vi "PatchCore_DS_Reader.vi"(4 "Read Options":T1={"Read Bads?"=TRUE, "Read GTs?"=TRUE, "Update. DS Stats?"=FALSE}, 6 "Good Unique Labels":string[](array[string])=["normal", "good", "OK"], 7 "PreProc_Options_in":T2={"DS_Name"="", "Input_Dims"={"C"=3, "H"=224, "W"=224}, "Cropping"={"Left"=0.0, "Top"=0.0, "Right"=1.0, "Bottom"=1.0}, "Interpolation Type"=1, "MultiStage_ReSample?"=TRUE, "Dataset_Stats"={"means"={"R"=0.19849297, "G"=0.18453708, "B"=0.19229858}, "stds"={"R"=0.22779399, "G"=0.21340185, "B"=0.19371489}}} {"Dataset_Stats"."stds"."R" format="%#_3g"; "Dataset_Stats"."stds"."G" format="%#_3g"; "Dataset_Stats"."stds"."B" format="%#_3g"; "Dataset_Stats"."means"."R" format="%#_3g"; "Dataset_Stats"."means"."G" format="%#_3g"; "Dataset_Stats"."means"."B" format="%#_3g"; "Interpolation Type" items=["Zero Order", "Bi-Linear", "Quadratic", "Cubic Spline"]}, 8 "error in":errorcluster, 10 "GT Folder Path":path, 11 "Folder Path":path) -> (0 "error out":errorcluster, 1 "PreProc_Options_out":T2={"DS_Name"="", "Input_Dims"={"C"=3, "H"=224, "W"=224}, "Cropping"={"Left"=0.0, "Top"=0.0, "Right"=1.0, "Bottom"=1.0}, "Interpolation Type"=1, "MultiStage_ReSample?"=TRUE, "Dataset_Stats"={"means"={"R"=0.19849297, "G"=0.18453708, "B"=0.19229858}, "stds"={"R"=0.22779399, "G"=0.21340185, "B"=0.19371489}}} {"Dataset_Stats"."stds"."R" format="%#_3g"; "Dataset_Stats"."stds"."G" format="%#_3g"; "Dataset_Stats"."stds"."B" format="%#_3g"; "Dataset_Stats"."means"."R" format="%#_3g"; "Dataset_Stats"."means"."G" format="%#_3g"; "Dataset_Stats"."means"."B" format="%#_3g"; "Interpolation Type" items=["Zero Order", "Bi-Linear", "Quadratic", "Cubic Spline"]}, 3 "Dataset":T7, 5 "dT_DS_Reader":dbl=1.5722605000046315)   [LabVIEW 2020]
uses:
  <vilib>/Ngene/Deep Learning Toolkit/Toolkit/NN_Data/API/DataSet/DataSet_Types/NN_DataSet(In3D_Out3D).ctl
  <vilib>/Ngene/Deep Learning Toolkit/Toolkit/NN_Data/API/NN_Dims(C,H,W).ctl
  <vilib>/Ngene/Deep Learning Toolkit/Toolkit/NN_Data/Controls/DataRef_Types/4D/NN_Data_ref(4D_SGL).ctl
  <vilib>/Ngene/DeepLTK Anomaly Detection Addon/Toolkit/API/Controls/NNPC_PreProcessing_Options.ctl
  <vilib>/Ngene/DeepLTK Anomaly Detection Addon/Toolkit/API/Controls/Crop_CFG.ctl
  <vilib>/Ngene/DeepLTK Anomaly Detection Addon/Toolkit/API/Controls/NNPC_DS_Stats.ctl
  <vilib>/Ngene/DeepLTK Anomaly Detection Addon/Toolkit/API/Controls/Image_Stats_RGB.ctl
  Controls/Read_Options.ctl
  <vilib>/Ngene/DeepLTK Anomaly Detection Addon/Toolkit/API/Controls/NNPC_DS_Custom_Data.ctl
  99e5ce4f-b18a-48c0-8340-627915dc1de5.vi
  39b6eea5-2cfc-4ae9-b230-8dd7afd04afa.vi
  <vilib>/Utility/High Resolution Relative Seconds.vi
  <vilib>/Ngene/Deep Learning Toolkit/Toolkit/Deep_Learning_Toolkit_by_Ngene.lvlib
  <vilib>/Ngene/DeepLTK Anomaly Detection Addon/Toolkit/DeepLTK_Anomaly_Detection_Addon.lvlib
  <vilib>/vision/NI_Vision_Development_Module.lvlib
panel:
  out "Progress":i32=41
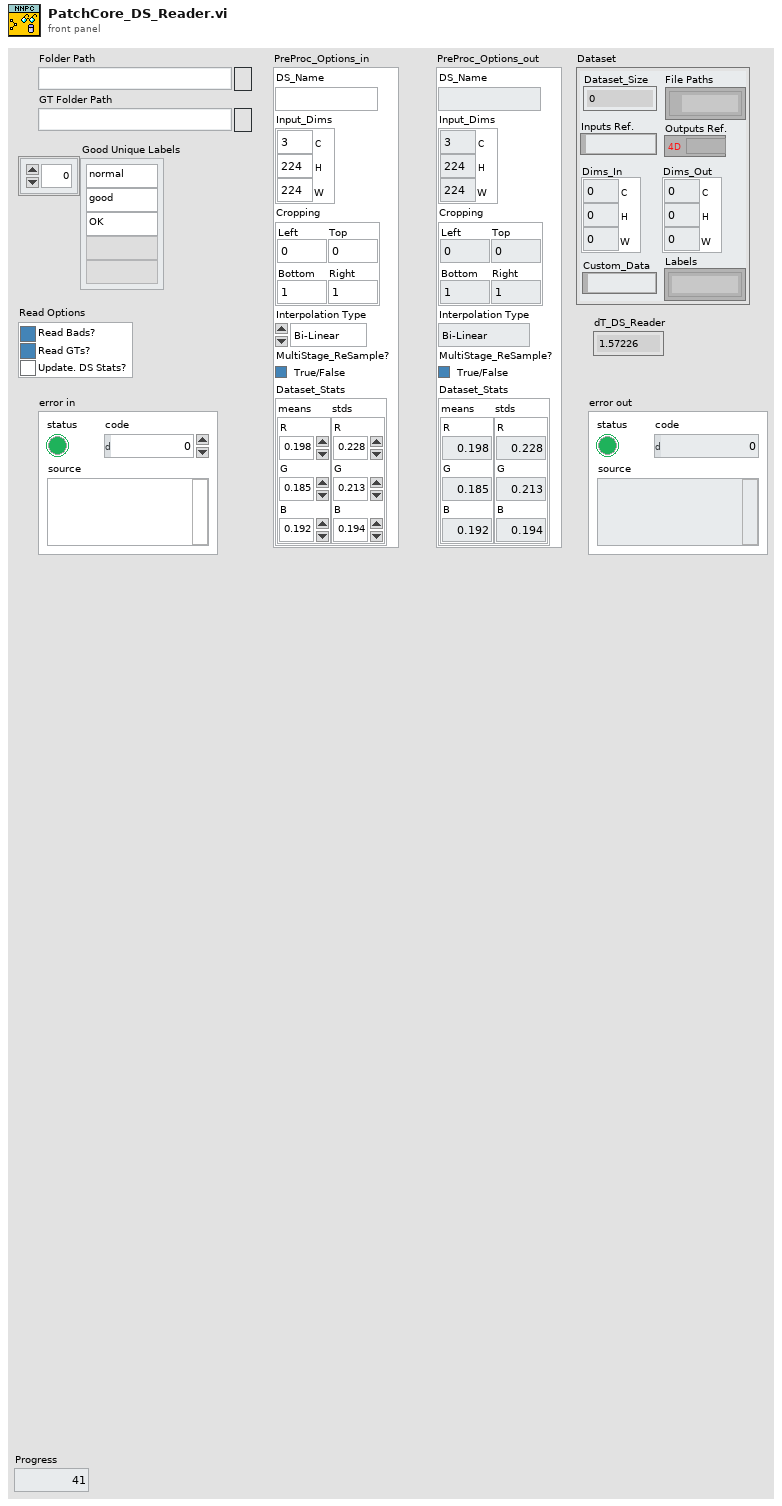
[diagram p1: front panel]
types:
  T1 = typedef "Read_Options.ctl" = cluster{"Read Bads?":bool, "Read GTs?":bool, "Update. DS Stats?":bool}
  T2 = typedef "DeepLTK_Anomaly_Detection_Addon.lvlib/NNPC_PreProcessing_Options.ctl" = cluster{"DS_Name":string, "Input_Dims":T3, "Cropping":T4, "Interpolation Type":u32, "MultiStage_ReSample?":bool, "Dataset_Stats":T5}
  T3 = typedef "Deep_Learning_Toolkit_by_Ngene.lvlib/NN_Dims(C,H,W).ctl" = cluster{"C":i32, "H":i32, "W":i32}
  T4 = typedef "DeepLTK_Anomaly_Detection_Addon.lvlib/Crop_CFG.ctl" = cluster{"Left":sgl, "Top":sgl, "Right":sgl, "Bottom":sgl}
  T5 = typedef "DeepLTK_Anomaly_Detection_Addon.lvlib/NNPC_DS_Stats.ctl" = cluster{"means":T6, "stds":T6}
  T6 = typedef "DeepLTK_Anomaly_Detection_Addon.lvlib/Image_Stats_RGB.ctl" = cluster{"R":sgl, "G":sgl, "B":sgl}
  T7 = typedef "Deep_Learning_Toolkit_by_Ngene.lvlib/NN_DataSet(In3D_Out3D).ctl" = cluster{"Dataset_Size":i32, "Dims_In":T3, "Labels":string[], "File Paths":path[], "Outputs Ref.":T8, "Inputs Ref.":variant, "Dims_Out":T3, "Custom_Data":variant}
  T8 = typedef "Deep_Learning_Toolkit_by_Ngene.lvlib/NN_Data_ref(4D_SGL).ctl" = refnum<data-value>
  T9 = typedef "DeepLTK_Anomaly_Detection_Addon.lvlib/NNPC_DS_Custom_Data.ctl" = cluster{"HasPixelGT?":bool, "ImageGT":refnum<data-value>, "PixelGT":refnum<data-value>}
  T10 = typedef "Image Type" = u32
  T11 = typedef "IMAQ Image.ctl" = refnum<image>
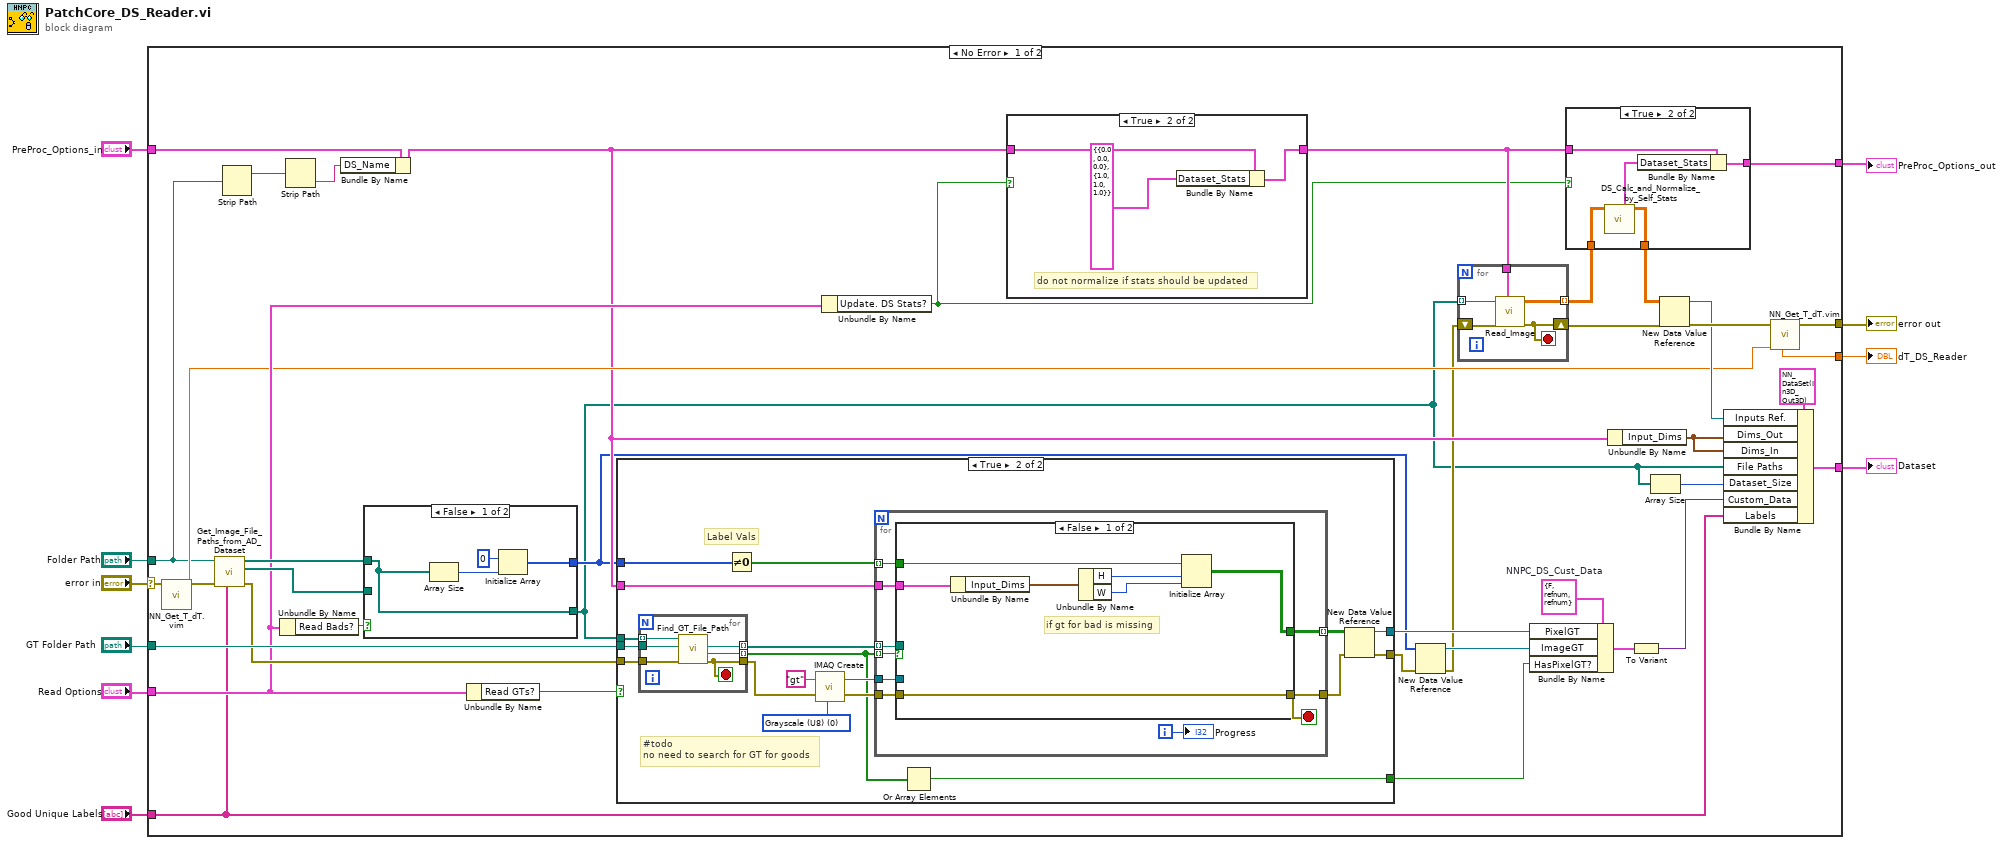
[diagram p0: block diagram]
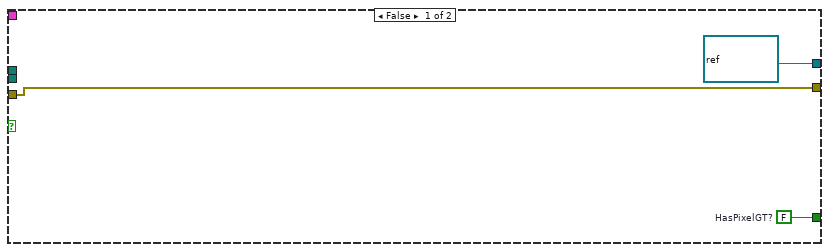
[diagram p2: hidden frame]
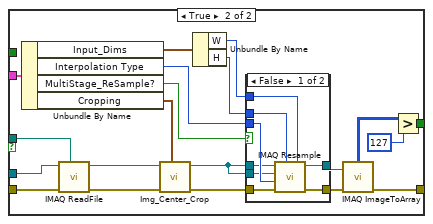
[diagram p3: hidden frame]
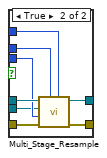
[diagram p4: hidden frame]
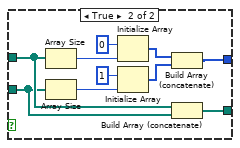
[diagram p5: hidden frame]
diagram:
  n1 = case shown="No Error" "error in" {
    selector: "error in" -> [w50 w160]
    tunnel: [w49 _] -> w9
    tunnel: "GT Folder Path" -> [w47 _]
    tunnel: "Good Unique Labels" -> [w19 _]
    tunnel: "Read Options" -> [w40 _]
    tunnel: [w37 w160] -> w5
    tunnel: [w35 _] -> w4
    tunnel: "Folder Path" -> [w34 _]
    tunnel: "PreProc_Options_in" -> [w31 _]
    tunnel: [w23 _] -> w1
    frame No Error {
      w22 = T9 {"HasPixelGT?"=FALSE, "ImageGT"=refnum, "PixelGT"=refnum}  # NNPC_DS_Cust_Data
      n2 = call "NN_Get_T_dT.vim"("error in"=w50) -> ("T_out"=w36:dbl, "error out"=w38:errorcluster)  [unwired: 6 in, 1 out]
      n3 = call "Get_Image_File_Paths_from_AD_Dataset.vi"("Good Folder Names"=w19, "error in"=w38, "Dataset Folder"=w34) -> ("error out"=w42:errorcluster, "Bad Dataset Files"=w45:path[], "Good Dataset Files"=w44:path[])  [unwired: 6 in]
      n4 = Strip Path(path=w34) -> (stripped path=w33:path)  [unwired: 1 out]
      n5 = Unbundle By Name(w40) -> ("Read Bads?"=w43:bool)
      n6 = Strip Path(path=w33) -> (name=w29:string)  [unwired: 1 out]
      n7 = Bundle By Name(cluster=w31, "DS_Name"=w29) -> (w30:T2)
      n8 = case shown="False" w43 {
        tunnel: w44 -> [w131 w142]
        tunnel: [w131 w143] -> w12
        tunnel: w45 -> [_ w137]
        tunnel: [w130 w134] -> w16
        frame False {
          n9 = Array Size(array=w131) -> (size(s)=w133:i32)
          n10 = Initialize Array(0 ("element"), w133) -> (w130:i32[])
        }
        frame True {
          n11 = Array Size(array=w142) -> (size(s)=w141:i32)
          n12 = Array Size(array=w137) -> (size(s)=w138:i32)
          n13 = Initialize Array(0 ("element"), w141) -> (w136:i32[])
          n14 = Initialize Array(1 ("element"), w138) -> (w135:i32[])
          n15 = Build Array (concatenate)(w136, w135) -> (w134:i32[])
          n16 = Build Array (concatenate)(w142, w137) -> (w143:path[])
        }
      }
      n17 = Unbundle By Name(w40) -> ("Read GTs?"=w20:bool)
      n18 = case shown="True" w20 {
        tunnel: w42 -> [w53 w64]
        tunnel: w47 -> [_ w66]
        tunnel: [w53 w54] -> w14
        tunnel: w12 -> [_ w65]
        tunnel: w16 -> [_ w59]
        tunnel: w30 -> [_ w62]
        tunnel: [refnum<data-value> refnum ("data value reference") w60] -> w17
        tunnel: [w51 w56] -> w11
        frame False {
          w51 = FALSE  # HasPixelGT?
        }
        frame True {
          w68 = T10 0 items=["Grayscale (U8)", "Grayscale (I16)", "Grayscale (SGL)", "Complex (CSG)", "RGB (U32)", "HSL (U32)", "RGB (U64)", "Grayscale (U16)"] ("Image Type")
          # "#todo\nno need to search for GT for goods"
          # "Label Vals"
          n19 = for {
            tunnel: w66 -> [w77]
            tunnel: w65 -> [w74] mode=indexing
            tunnel: [w75] -> w67 mode=indexing
            tunnel: [w76] -> w57 mode=indexing
            tunnel: w64 -> [w73]
            tunnel: [w72] -> w63
            stop <- w72 stop-if-true
            n20 = call "Find_GT_File_Path.vi"("error in"=w73, "GT Mask Folder Path"=w77, "Image File Path"=w74) -> ("error out"=w72:errorcluster, "Found?"=w76:bool, "GT File Path"=w75:path)  [unwired: 5 in, 1 out]
          }
          n21 = Not Equal To 0?(x=w59) -> (x != 0?=w58:bool[])
          n22 = call "IMAQ Create"("Image Name"="gt", "Image Type"=w68, "error in (no error)"=w63) -> ("New Image"=w71:T11, "error out"=w69:errorcluster)  [unwired: 2 in]
          n23 = for {
            tunnel: w71 -> [w86]
            tunnel: w67 -> [w84] mode=indexing
            tunnel: w57 -> [w81] mode=indexing
            tunnel: w58 -> [w80] mode=indexing
            tunnel: w62 -> [w79]
            tunnel: [w78] -> w61 mode=indexing
            tunnel: w69 -> [w85]
            tunnel: [w82] -> w55
            i -> [w83]
            stop <- w82 stop-if-true
            n24 = case shown="False" w81 {
              tunnel: w86 -> [_ w113]
              tunnel: w85 -> [w93 w112]
              tunnel: w84 -> [_ w111]
              tunnel: [w93 w110] -> w82
              tunnel: w80 -> [w90 _]
              tunnel: w79 -> [w88 w108]
              tunnel: [w87 w105] -> w78
              frame False {
                # "if gt for bad is missing"
                n25 = Unbundle By Name(w88) -> ("Input_Dims"=w89:T3)
                n26 = Unbundle By Name(w89) -> ("H"=w91:i32, "W"=w92:i32)
                n27 = Initialize Array(w90, w91, w92) -> (w87:bool[][])
              }
              frame True {
                n28 = Unbundle By Name(w108) -> ("Input_Dims"=w109:T3, "Interpolation Type"=w99:u32, "MultiStage_ReSample?"=w98:bool, "Cropping"=w102:T4)
                n29 = call "IMAQ ReadFile"("File Path"=w111, "error in (no error)"=w112, "Image"=w113) -> ("error out"=w103:errorcluster, "Image Out"=w104:T11)  [unwired: 4 in, 3 out]
                n30 = call "Img_Center_Crop.vi"("Crop_CFG"=w102, "error in"=w103, "Image Src In"=w104) -> ("error out"=w95:errorcluster, "Image Dest Out"=w94:T11)  [unwired: 7 in]
                n31 = Unbundle By Name(w109) -> ("W"=w100:i32, "H"=w101:i32)
                n32 = case shown="False" w98 {
                  tunnel: [w121 w126] -> w96
                  tunnel: [w120 w127] -> w97
                  tunnel: w99 -> [w119 w123]
                  tunnel: w94 -> [w115 w124]
                  tunnel: w100 -> [w118 w125]
                  tunnel: w101 -> [w117 w128]
                  tunnel: w95 -> [w116 w129]
                  tunnel: w94 -> [w114 w122]
                  frame False {
                    n33 = call "IMAQ Resample"("X Resolution"=w118, "Y Resolution"=w117, "error in (no error)"=w116, "Interpolation Type"=w119, "Image Dst"=w114, "Image Src"=w115) -> ("error out"=w121:errorcluster, "Image Dst Out"=w120:T11)  [unwired: 4 in]
                  }
                  frame True {
                    n34 = call "Multi_Stage_Resample.vi"("X Resolution"=w125, "Y Resolution"=w128, "error in"=w129, "Interpolation Type"=w123, "Image Dest In"=w122, "Image Src"=w124) -> ("error out"=w126:errorcluster, "Img out"=w127:T11)  [unwired: 4 in]
                  }
                }
                n35 = call "IMAQ ImageToArray"("error in (no error)"=w96, "Image"=w97) -> ("error out"=w110:errorcluster, "Image Pixels (U8)"=w107:u8[][])  [unwired: 2 in, 3 out]
                n36 = Greater?(x=w107, y=u8 127) -> (0:w105:bool[][])
              }
            }
            "Progress" <- w83
          }
          n37 = Or Array Elements(Boolean array=w57) -> (logical OR=w56:bool)
          n38 = New Data Value Reference(data value=w61, error in=w55) -> (data value reference=w60:refnum<data-value>, error out=w54:errorcluster)
        }
      }
      n39 = Unbundle By Name(w40) -> ("Update. DS Stats?"=w24:bool)
      n40 = case shown="True" w24 {
        tunnel: w30 -> [w144 w147]
        tunnel: [w144 w145] -> w26
        frame False {
        }
        frame True {
          # "do not normalize if stats should be updated"
          n41 = Bundle By Name(cluster=w147, "Dataset_Stats"=T5 {"means"={"R"=0.0, "G"=0.0, "B"=0.0}, "stds"={"R"=1.0, "G"=1.0, "B"=1.0}}) -> (w145:T2)
        }
      }
      n42 = New Data Value Reference(data value=w16, error in=w14) -> (data value reference=w15:refnum<data-value>, error out=w13:errorcluster)
      n43 = for {
        tunnel: [w148] -> w27 mode=indexing
        tunnel: w26 -> [w149]
        tunnel: w12 -> [w150] mode=indexing
        shift-right: [w151] -> w28
        shift-left: w13 -> [w152]
        stop <- w151 stop-if-true
        n44 = call "Read_Image.vi"("PreProcessing_Options"=w149, "error in"=w152, "Img Path"=w150) -> ("error out"=w151:errorcluster, "Image Out (Preproc)"=w148:sgl[][][])  [unwired: 3 in, 4 out]
      }
      n45 = Bundle By Name(cluster=w22, "PixelGT"=w17, "ImageGT"=w15, "HasPixelGT?"=w11) -> (w18:T9)
      n46 = case shown="True" w24 {
        tunnel: w27 -> [w154 w157]
        tunnel: [w154 w155] -> w25
        tunnel: w26 -> [w153 w159]
        tunnel: [w153 w158] -> w23
        frame False {
        }
        frame True {
          n47 = call "DS_Calc_and_Normalize_by_Self_Stats.vi"("DS in"=w157) -> ("DS out"=w155:sgl[][][][], "Dataset_Stats"=w156:T5)  [unwired: 9 in]
          n48 = Bundle By Name(cluster=w159, "Dataset_Stats"=w156) -> (w158:T2)
        }
      }
      n49 = Unbundle By Name(w30) -> ("Input_Dims"=w32:T3)
      n50 = To Variant(anything=w18) -> (Variant=w21:variant)
      n51 = Array Size(array=w12) -> (size(s)=w39:i32)
      n52 = New Data Value Reference(data value=w25, error in=w28) -> (data value reference=w41:refnum<data-value>, error out=w46:errorcluster)
      n53 = Bundle By Name(cluster=T7 {"Dataset_Size"=0, "Dims_In"={"C"=0, "H"=0, "W"=0}, "Labels"=[], "File Paths"=[], "Outputs Ref."=refnum, "Inputs Ref."=variant, "Dims_Out"={"C"=0, "H"=0, "W"=0}, "Custom_Data"=variant} ("Dataset(In3D_Out3D)"), "Inputs Ref."=w41, "Dims_Out"=w32, "Dims_In"=w32, "File Paths"=w12, "Dataset_Size"=w39, "Custom_Data"=w21, "Labels"=w19) -> (w49:T7)
      n54 = call "NN_Get_T_dT.vim"("T_in"=w36, "error in"=w46) -> ("error out"=w37:errorcluster, "dT"=w35:dbl)  [unwired: 5 in, 1 out]
    }
    frame Error {
    }
  }
  "error out" <- w5
  "Dataset" <- w9
  "dT_DS_Reader" <- w4
  "PreProc_Options_out" <- w1
